vi "set Frequency Line.vi"(8 "error in (no error)":errorcluster, 10 "Frequency Line (Hz)":T1 {"Line 2" format="%#_6p"; "Line 1" format="%#_6p"}, 11 "Keysight 9020A in":refnum<class "Keysight 9020A.lvclass">) -> (0 "error out":errorcluster, 3 "Keysight 9020A out":refnum<class "Keysight 9020A.lvclass">)   [LabVIEW 2023, in "Spectrum Analyzer.lvlib" / "Keysight 9020A.lvclass"]
uses:
  Keysight 9020A.lvclass
  TYPE DEFINITION/TYPE Frequency Line Param.ctl
  Keysight 9020A.lvclass/Keysight 9020A.ctl
  Spectrum Analyzer.lvlib
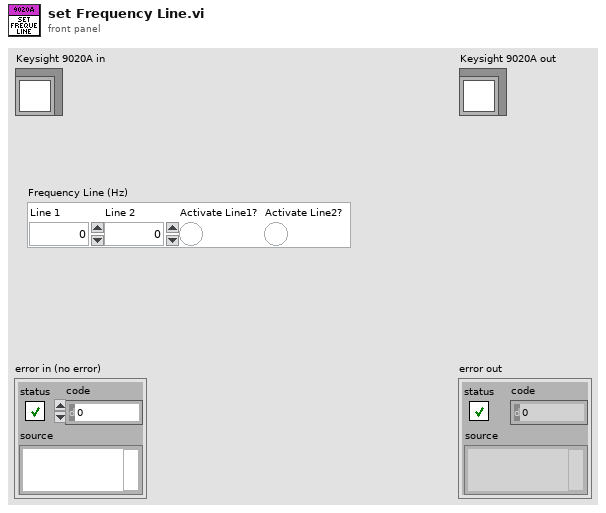
[diagram p1: front panel]
types:
  T1 = typedef "Spectrum Analyzer.lvlib/TYPE Frequency Line Param.ctl" = cluster{"Line 1":dbl, "Line 2":dbl, "Activate Line1?":bool, "Activate Line2?":bool}
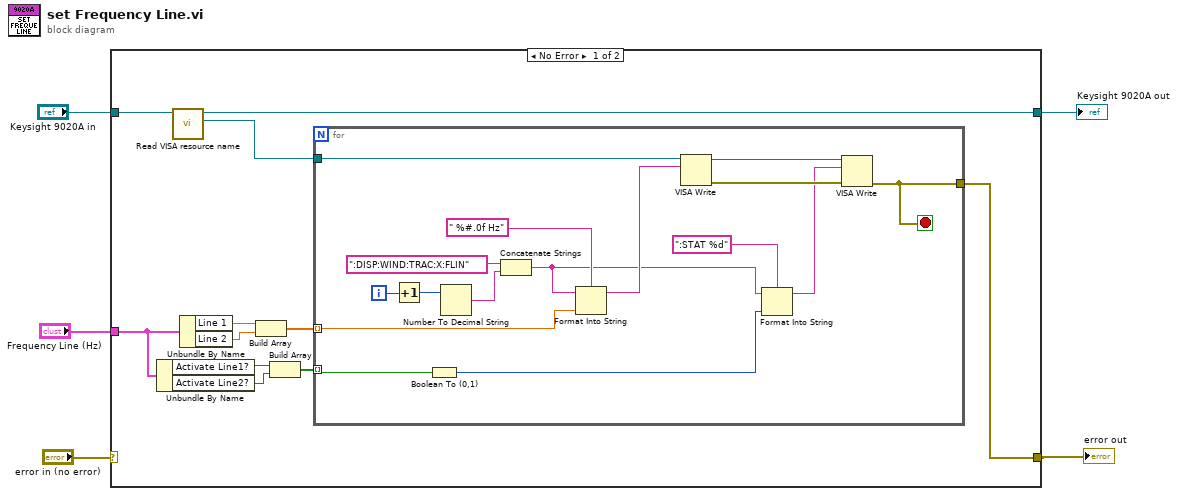
[diagram p0: block diagram]
diagram:
  n1 = case shown="No Error" "error in (no error)" {
    selector: "error in (no error)" -> [_ w33]
    tunnel: "Keysight 9020A in" -> [w16 w34]
    tunnel: [w15 w34] -> w4
    tunnel: [w6 w33] -> w2
    tunnel: "Frequency Line (Hz)" -> [w10 _]
    frame No Error {
      n2 = Unbundle By Name(w10) -> ("Activate Line1?"=w9:bool, "Activate Line2?"=w8:bool)
      n3 = call "Read VISA resource name.vi"("Keysight 9020A in"=w16) -> ("VISA resource name"=w14:refnum<visa-resource-name>, "Keysight 9020A out"=w15:refnum<class "Keysight 9020A.lvclass">)  [unwired: 8 in, 1 out]
      n4 = Unbundle By Name(w10) -> ("Line 1"=w13:dbl, "Line 2"=w12:dbl)
      n5 = Build Array(w13, w12) -> (w11:dbl[])
      n6 = Build Array(w9, w8) -> (w7:bool[])
      n7 = for {
        tunnel: w14 -> [w32]
        tunnel: w11 -> [w25] mode=indexing
        tunnel: w7 -> [w22] mode=indexing
        tunnel: [w18] -> w6
        i -> [w29]
        stop <- w18 stop-if-true
        n8 = Increment(x=w29) -> (x+1=w28:i32)
        n9 = Boolean To (0,1)(Boolean=w22) -> (0, 1=w21:i16)
        n10 = Number To Decimal String(number=w28) -> (decimal integer string=w26:string)  [unwired: 1 in]
        n11 = Concatenate Strings(":DISP:WIND:TRAC:X:FLIN", w26) -> (w24:string)
        n12 = Format Into String(format string=" %#.0f Hz", initial string=w24, w25) -> (resulting string=w31:string)  [unwired: 1 in, 1 out]
        n13 = VISA Write(VISA resource name=w32, write buffer=w31) -> (VISA resource name out=w20:refnum<visa-resource-name>, error out=w19:errorcluster)  [unwired: 1 in, 1 out]
        n14 = Format Into String(format string=":STAT %d", initial string=w24, w21) -> (resulting string=w17:string)  [unwired: 1 in, 1 out]
        n15 = VISA Write(VISA resource name=w20, write buffer=w17, error in (no error)=w19) -> (error out=w18:errorcluster)  [unwired: 2 out]
      }
    }
    frame Error {
    }
  }
  "error out" <- w2
  "Keysight 9020A out" <- w4
